vi "Wyznaczanie THD.vi"() -> ()   [LabVIEW 2026]
panel:
  in  "stop":bool
  out "THD [%]":dbl
  out "Wykres":dbl[](graph)
  in  "Faza [deg]":dbl(knob) scale=0.0..360.0
  in  "Czêstotliwoœæ [Hz]":dbl(knob) scale=0.0..10.0
  in  "Amplituda 1h":dbl(knob) scale=0.0..100.0
  in  "Amplituda 3h":dbl(knob) scale=0.0..100.0
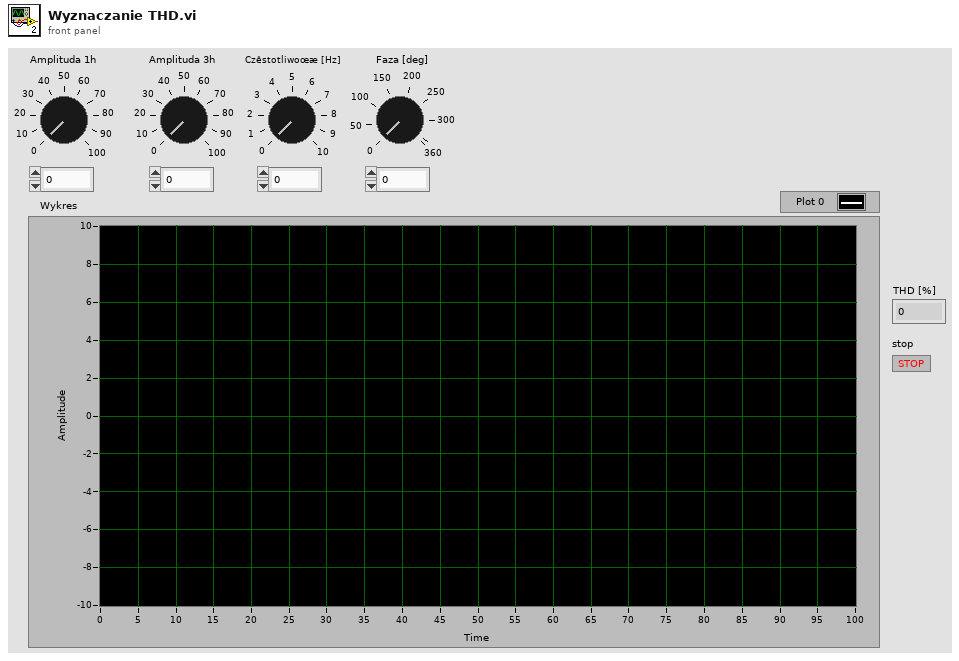
[diagram p1: front panel]
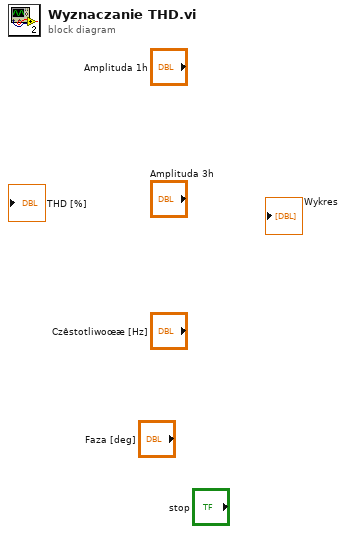
[diagram p0: block diagram]
diagram:
